vi "Split DMA by Direction.vi"(8 "error in":errorcluster, 11 "DMA configuration array":T1[](array[typedef])) -> (0 "error out":errorcluster, 2 "HostToTarget":T4[](array[typedef]) {"Data Type" format="%.0x"}, 3 "TargetToHost":T4[](array[typedef]) {"Data Type" format="%.0x"})   [LabVIEW 2019, in "FPGA Addon System Explorer.lvlib"]
uses:
  FPGA Addon System Explorer.lvlib
  Addon Shared/Types/DMA Information.ctl
  Addon Shared/Types/Data Type.ctl
  <vilib>/rvi/FIFO/Fifo_Types/Fifo_DMA_Config.ctl
  <vilib>/rvi/DataTransferAndStorage/Container/Common/niFpgaDataTypeControl.ctl
  <vilib>/rvi/ClientSDK/Core/ModuleGeneration/CommunicationInterfaceUtility/niFpgaDmaChannelImplementation.ctl
  Addon Shared/FPGA Addon Shared.lvlib
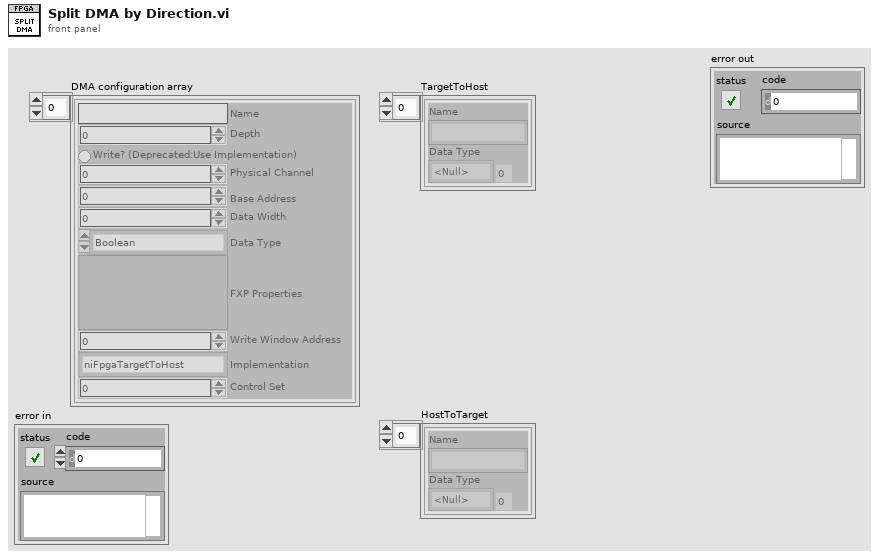
[diagram p1: front panel]
types:
  T1 = typedef "Fifo_DMA_Config.ctl" = cluster{"Name":string, "Depth":u32, "Write? (Deprecated:Use Implementation)":bool, "Physical Channel":u32, "Base Address":u32, "Data Width":u32, "Data Type":T2, "FXP Properties":variant, "Write Window Address":u32, "Implementation":T3, "Control Set":u32}
  T2 = typedef "niFpgaDataTypeControl.ctl" = enum32{"Boolean", "I8", "I16", "I32", "I64", "U8", "U16", "U32", "U64", "FXP", "CustomControl", "SGL"}
  T3 = typedef "niFpgaDmaChannelImplementation.ctl" = enum16{"niFpgaTargetToHost", "niFpgaHostToTarget", "niFpgaPeerToPeerWriter", "niFpgaPeerToPeerReader", "niCoreTargetToHost", "niCoreHostToTarget"}
  T4 = typedef "FPGA Addon Shared.lvlib/DMA Information.ctl" = cluster{"Name":string, "Data Type":T5}
  T5 = typedef "FPGA Addon Shared.lvlib/Data Type.ctl" = enum8{"<Null>", "I8", "I16", "I32", "I64", "U8", "U16", "U32", "U64", "SGL", "Boolean", "Analog PWM In Settings", "Analog PWM In", "Digital PWM In Settings", "Digital PWM In", "Digital PWM Out", "Sine Out", "FXP+/-24.5", "FXP+/-16.5", "FXP+/-32.8", "FXP+/-64.32", "FXP+/-16.7", "FXP+/-20.5", "FXP+/-27.5", "FXP+/-32.16", "FXP +16.3", "FXP +18.3", "Digital Static In", "Digital Static Out", "Digital Static In Settings", "Digital WSS Out", "Quad Encoder Settings", "Quad Encoder In"}
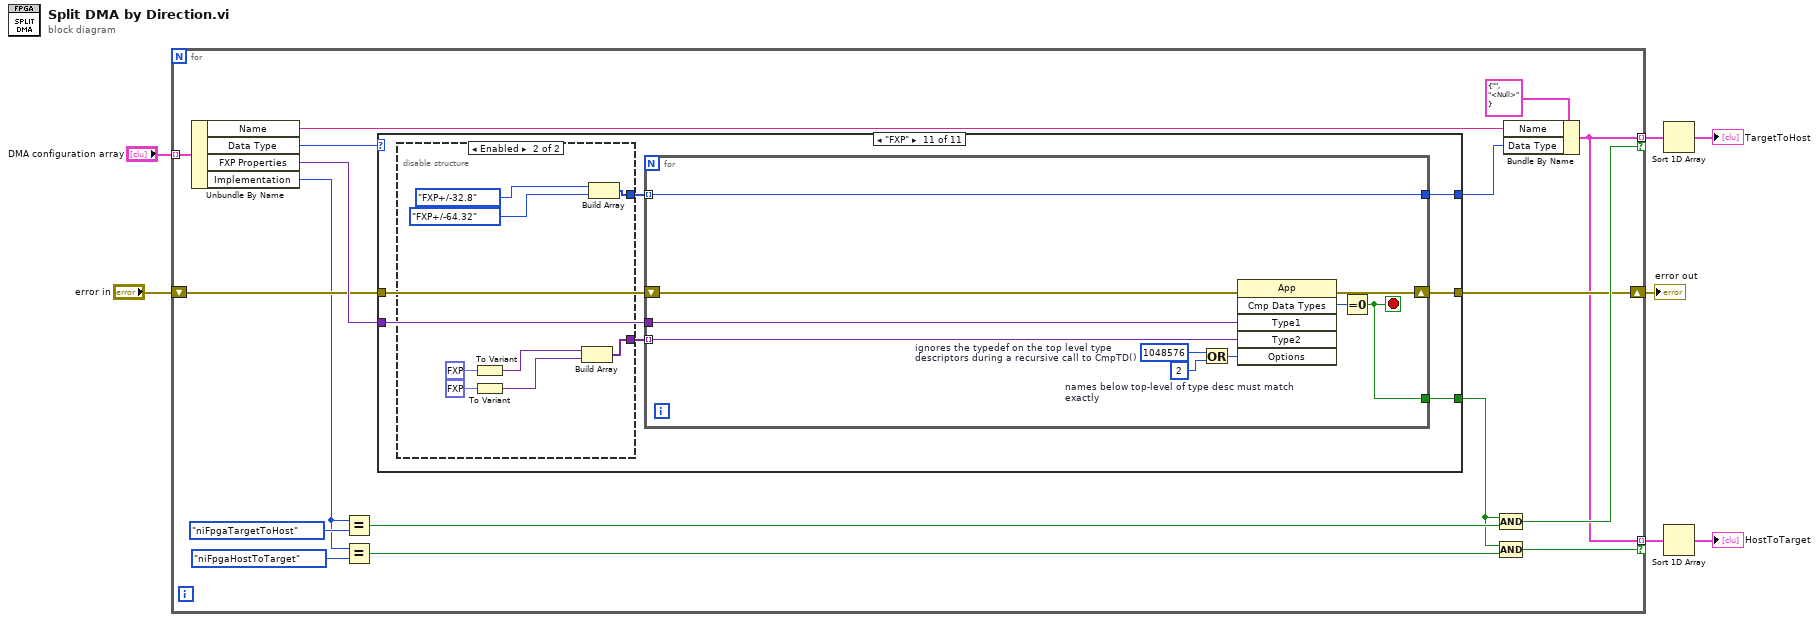
[diagram p0: block diagram]
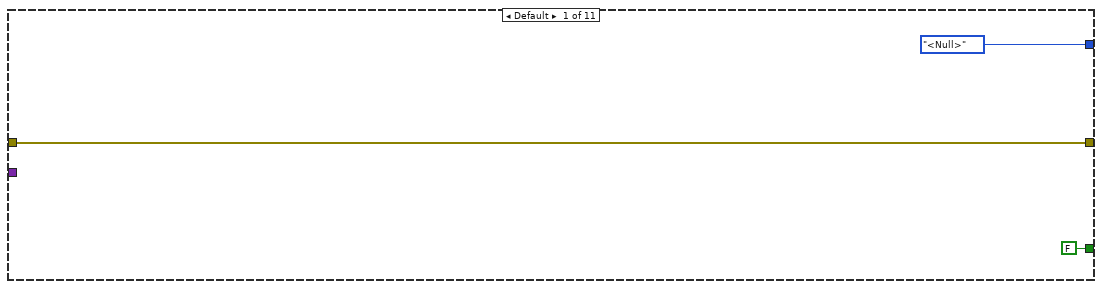
[diagram p2: hidden frame]
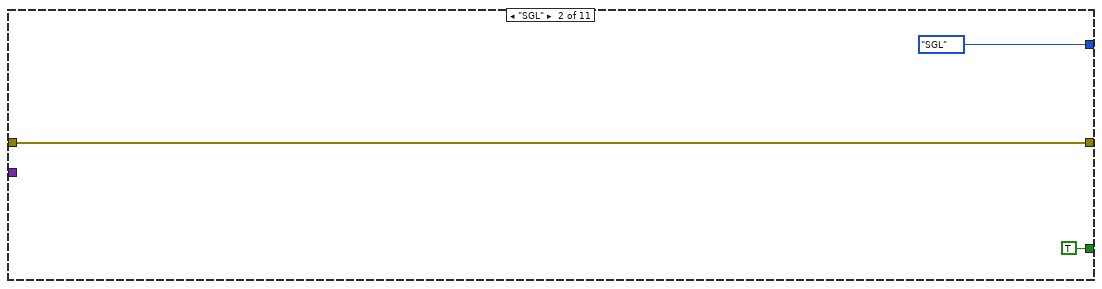
[diagram p3: hidden frame]
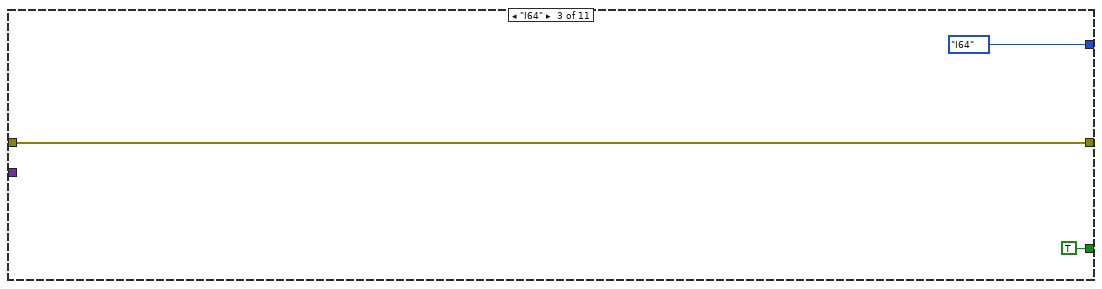
[diagram p4: hidden frame]
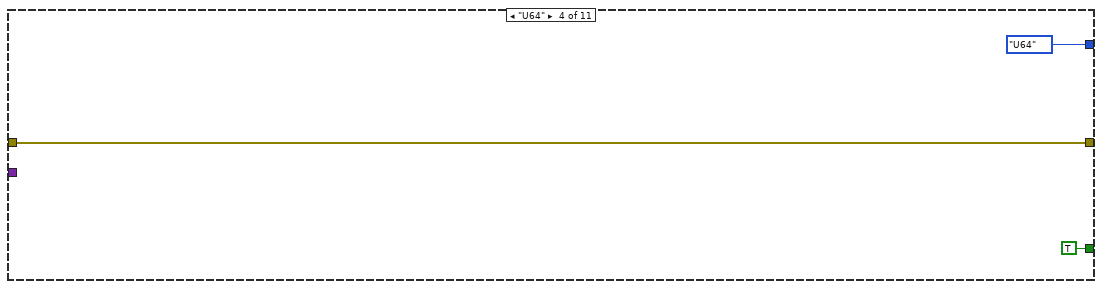
[diagram p5: hidden frame]
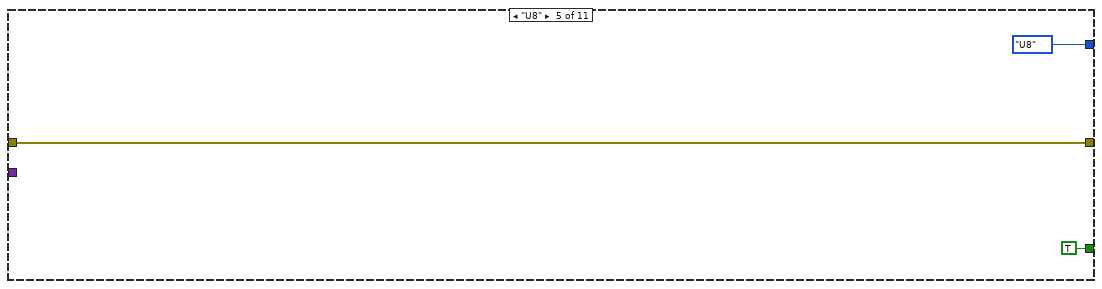
[diagram p6: hidden frame]
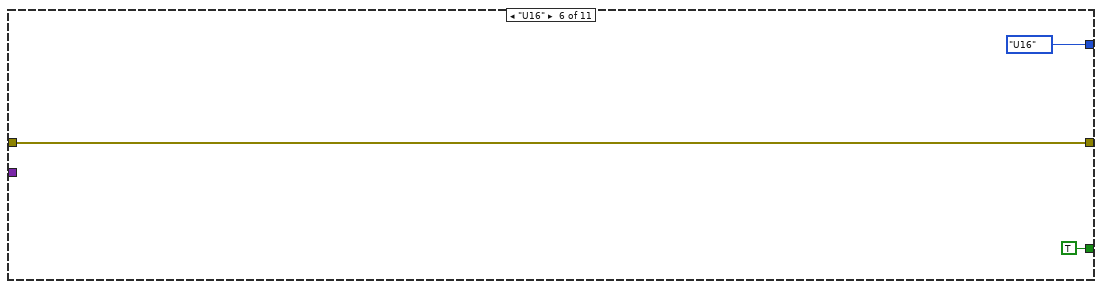
[diagram p7: hidden frame]
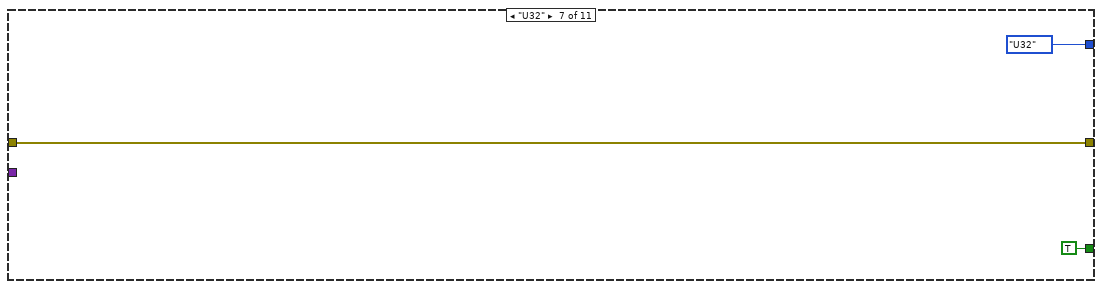
[diagram p8: hidden frame]
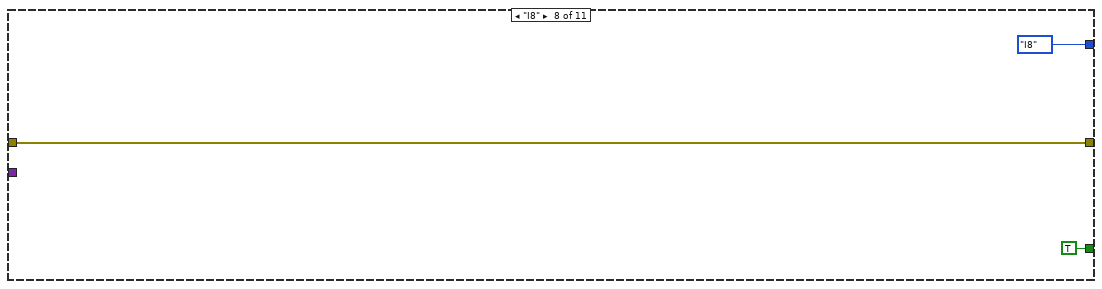
[diagram p9: hidden frame]
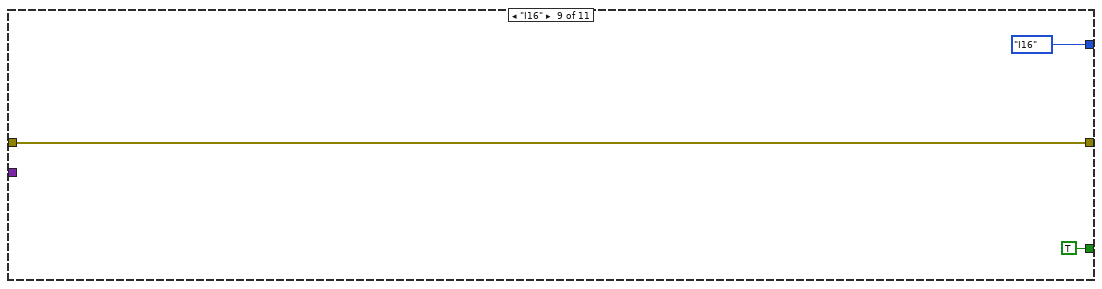
[diagram p10: hidden frame]
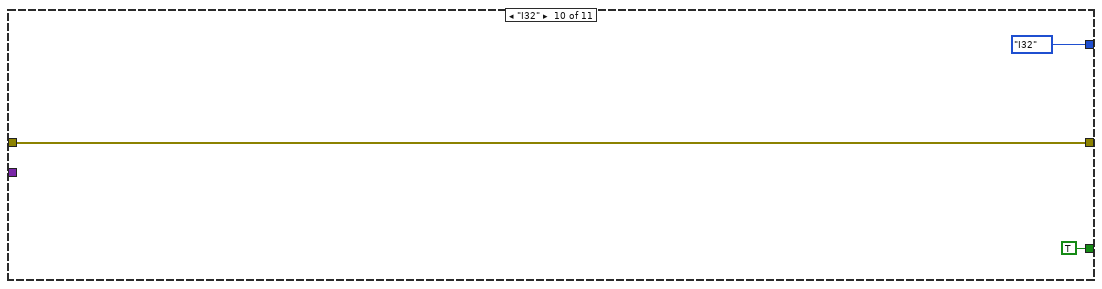
[diagram p11: hidden frame]
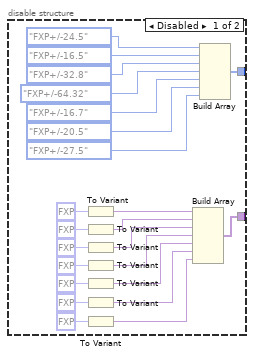
[diagram p12: hidden frame]
diagram:
  n1 = for {
    tunnel: "DMA configuration array" -> [w10] mode=indexing
    tunnel: [w9] -> w3 mode=indexing if=w21
    tunnel: [w9] -> w5 mode=indexing if=w19
    shift-right: [w17] -> w2
    shift-left: "error in" -> [w16]
    n2 = Unbundle By Name(w10) -> ("Name"=w14:string, "Data Type"=w13:T2, "FXP Properties"=w18:variant, "Implementation"=w8:T3)
    n3 = Equal?(x=w8, y=niFpgaDmaChannelImplementation."niFpgaTargetToHost") -> (x = y?=w22:bool)
    n4 = Equal?(x=w8, y=niFpgaDmaChannelImplementation."niFpgaHostToTarget") -> (x = y?=w20:bool)
    n5 = case shown="\"FXP\"" w13 {
      tunnel: w18 -> [_ _ _ _ _ _ _ _ _ _ w61]
      tunnel: [w27 w30 w33 w36 w39 w42 w45 w48 w51 w54 w60] -> w17
      tunnel: w16 -> [w27 w30 w33 w36 w39 w42 w45 w48 w51 w54 w59]
      tunnel: [Data_Type."<Null>" ("Data Type") Data_Type."SGL" ("Data Type") Data_Type."I64" ("Data Type") Data_Type."U64" ("Data Type") Data_Type."U8" ("Data Type") Data_Type."U16" ("Data Type") Data_Type."U32" ("Data Type") Data_Type."I8" ("Data Type") Data_Type."I16" ("Data Type") Data_Type."I32" ("Data Type") w56] -> w12
      tunnel: [FALSE TRUE TRUE TRUE TRUE TRUE TRUE TRUE TRUE TRUE w55] -> w11
      frame Default {
      }
      frame "SGL" {
      }
      frame "I64" {
      }
      frame "U64" {
      }
      frame "U8" {
      }
      frame "U16" {
      }
      frame "U32" {
      }
      frame "I8" {
      }
      frame "I16" {
      }
      frame "I32" {
      }
      frame "FXP" {
        n6 = disable-structure shown="Enabled" {
          disable-tunnel: [w70 w88] -> w58
          disable-tunnel: [w62 w85] -> w57
          frame Disabled {
            n7 = To Variant(anything=fxp<+/-,24,5> 0.0 ("Numeric 1 In")) -> (Variant=w71:variant)
            n8 = To Variant(anything=fxp<+/-,16,5> 0.0 ("Numeric 2 In")) -> (Variant=w72:variant)
            n9 = To Variant(anything=fxp<+/-,32,8> 0.0 ("Numeric 3 In")) -> (Variant=w73:variant)
            n10 = To Variant(anything=fxp<+/-,64,32> 0.0 ("Numeric 4 In")) -> (Variant=w74:variant)
            n11 = To Variant(anything=fxp<+/-,16,7> 0.0 ("Numeric 4 In")) -> (Variant=w80:variant)
            n12 = To Variant(anything=fxp<+/-,20,5> 0.0 ("Numeric 4 In")) -> (Variant=w82:variant)
            n13 = To Variant(anything=fxp<+/-,27,5> 0.0 ("Numeric 4 In")) -> (Variant=w84:variant)
            n14 = Build Array(w71, w72, w73, w74, w80, w82, w84) -> (w70:variant[])
            n15 = Build Array(Data_Type."FXP+/-24.5" ("Data Type"), Data_Type."FXP+/-16.5" ("Data Type"), Data_Type."FXP+/-32.8" ("Data Type"), Data_Type."FXP+/-64.32" ("Data Type"), Data_Type."FXP+/-16.7" ("Data Type"), Data_Type."FXP+/-20.5" ("Data Type"), Data_Type."FXP+/-27.5" ("Data Type")) -> (w62:T5[])
          }
          frame Enabled {
            n16 = To Variant(anything=fxp<+/-,32,8> 0.0 ("Numeric 3 In")) -> (Variant=w89:variant)
            n17 = To Variant(anything=fxp<+/-,64,32> 0.0 ("Numeric 4 In")) -> (Variant=w90:variant)
            n18 = Build Array(w89, w90) -> (w88:variant[])
            n19 = Build Array(Data_Type."FXP+/-32.8" ("Data Type"), Data_Type."FXP+/-64.32" ("Data Type")) -> (w85:T5[])
          }
        }
        n20 = for {
          tunnel: w61 -> [w98]
          tunnel: w58 -> [w97] mode=indexing
          shift-right: [w96] -> w60
          shift-left: w59 -> [w95]
          tunnel: w57 -> [w94] mode=indexing
          tunnel: [w94] -> w56
          tunnel: [w93] -> w55
          stop <- w93 stop-if-true
          w99 = 2  # names below top-level of type desc must match exactly
          w101 = 1048576  # ignores the typedef on the top level type descriptors during a recursive call to CmpTD()
          n21 = Or(x=w101, y=w99) -> (x .or. y?=w102:i32)
          n22 = invoke class="App" method="Cmp Data Types"(error in=w95, "Type1"=w98, "Type2"=w97, "Options"=w102) -> (error out=w96:errorcluster, "Compare Data Types"=w100:i32)  [unwired: 2 in, 4 out]
          n23 = Equal To 0?(x=w100) -> (x = 0?=w93:bool)
        }
      }
    }
    n24 = Compound Arithmetic op=AND(w11, w22) -> (w21:bool)
    n25 = Compound Arithmetic op=AND(w11, w20) -> (w19:bool)
    n26 = Bundle By Name(cluster=T4 {"Name"="", "Data Type"=enum."<Null>"} ("Cluster"), "Name"=w14, "Data Type"=w12) -> (w9:T4)
  }
  "error out" <- w2
  n27 = Sort 1D Array(array=w3) -> (sorted array=→"TargetToHost":T4[])
  n28 = Sort 1D Array(array=w5) -> (sorted array=→"HostToTarget":T4[])
